vi "Checkpoint_Write.vi"(8 "error in (no error)":errorcluster={"status"=FALSE, "code"=0, "source"="\"\""}, 10 "result commit marker":string, 11 "RunContext":string) -> (0 "error out":errorcluster={"status"=FALSE, "code"=0, "source"="\"\""}, 2 "status ok":bool, 3 "Checkpoint receipt":string)   [LabVIEW 2026]
doc: "INTENT: Persist durable cycle boundary. LOGIC: Write version/run/cycle/checksum to temp file, flush and atomically replace per supported filesystem policy."
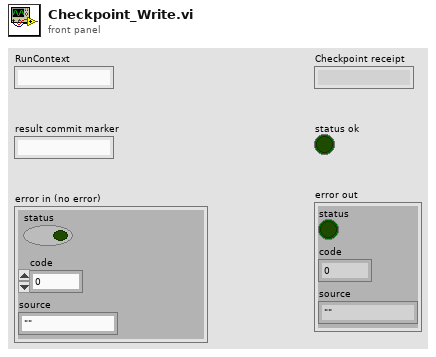
[diagram p1: front panel]
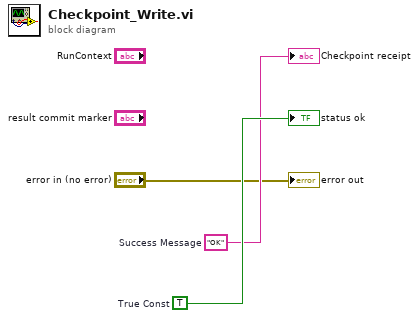
[diagram p0: block diagram]
diagram:
  w3 = TRUE  # True Const
  w2 = "OK"  # Success Message
  "Checkpoint receipt" <- w2
  "status ok" <- w3
  "error out" <- "error in (no error)"
